vi "Get Item Icon.vi"(8 "error in (no error)":errorcluster, 11 "VI in":refnum<class "VI.lvclass">) -> (0 "error out":errorcluster, 3 "VI out":refnum<class "VI.lvclass">)   [LabVIEW 2020, in "VI Properties Editor.lvlib" / "VI.lvclass"]
doc: "Gets the icon for <B>VI in</B>."
uses:
  VI.lvclass
  VI.lvclass/VI.ctl
  <vilib>/LabVIEW Icon API/lv_icon/Controls/Alignment.ctl
  <vilib>/LabVIEW Icon API/lv_icon/Controls/Font.ctl
  <vilib>/LabVIEW Icon API/lv_icon/Controls/BodyText.ctl
  <vilib>/LabVIEW Icon API/lv_icon/lv_icon.lvlib
  <vilib>/LabVIEW Icon API/LabVIEW Icon API.lvlib
  VI Properties Editor.lvlib
panel:
  in  "Localized string template":string="Template"
  in  "Localied string text":string="Text"
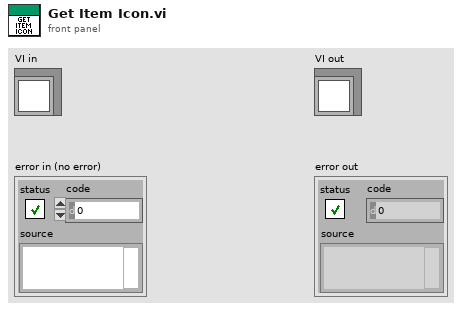
[diagram p1: front panel]
types:
  T1 = typedef "Font.ctl" = string
  T2 = typedef "BodyText.ctl" = cluster{"Line 1 text":string, "Line 2 text":string, "Line 3 text":string, "Line 4 text":string, "Line 1 color":u32, "Line 2 color":u32, "Line 3 color":u32, "Line 4 color":u32, "Body Text Spec":cluster{"Font":T1, "Alignment":T3, "Size":u8}, "Center text vertically":bool, "Capitalize Text":bool}
  T3 = typedef "Alignment.ctl" = u16
  T4 = typedef "LabVIEW Icon Stored Information.ctl" = cluster{"Text Visible?":bool, "Text Opacity":u8, "Templ Visible?":bool, "Templ Opacity":u8, "Relative Path from 1 to 2":path, "Image":picture, "All User Layers":refnum<class "Layer.lvclass">[], "Body Text":T2}
  T5 = typedef "imagedata.ctl" = cluster{"image type":i32, "image depth":i32, "image":u8[], "mask":u8[], "colors":u32[], "Rectangle":cluster{"left":i16, "top":i16, "right":i16, "bottom":i16}}
  T6 = typedef "Layer.ctl" = cluster{"LayerIcon":picture, "LayerName":string, "Opacity":u8, "Visibility?":bool}
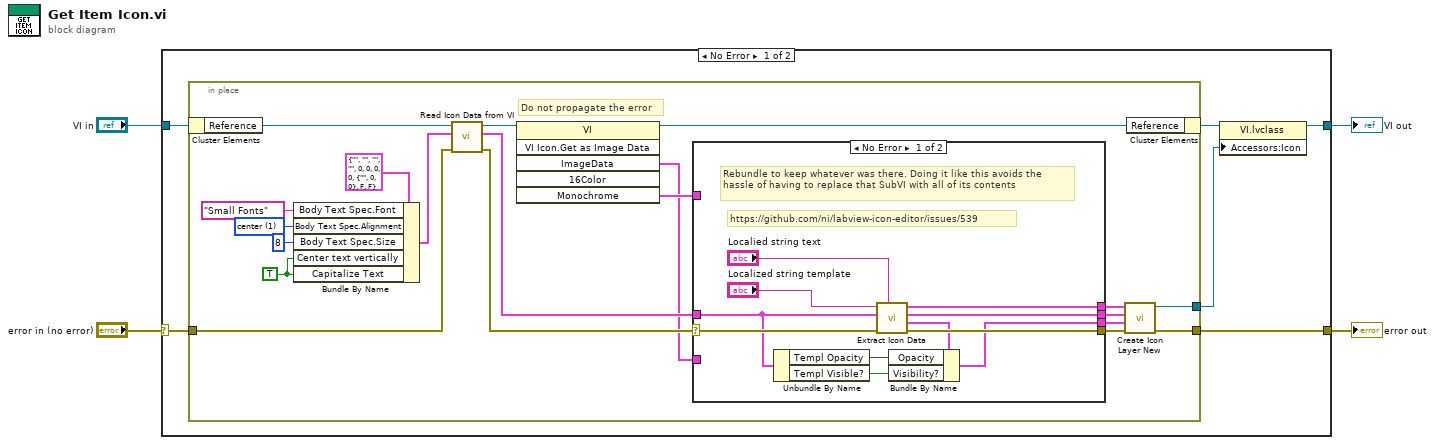
[diagram p0: block diagram]
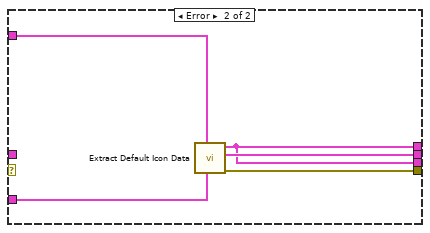
[diagram p2: hidden frame]
diagram:
  n1 = case shown="No Error" "error in (no error)" {
    selector: "error in (no error)" -> [w9 w46]
    tunnel: "VI in" -> [w10 w47]
    tunnel: [w8 w46] -> w2
    tunnel: [w5 w47] -> w1
    frame No Error {
      n2 = in-place {
        in-place-border: w9 -> [w28]
        in-place-border: [w18] -> w8
        in-place-border: [w17] -> w6
        w12 = TRUE ("Center text vertically")
        w14 = T3 1 items=["left", "center", "right"] ("Body Text Spec.Alignment")
        # "Do not propagate the error"
        n3 = in-place-cluster #1(w10) -> ("Reference"=w30:refnum<vi>)
        n4 = Bundle By Name(cluster=T2 {"Line 1 text"="", "Line 2 text"="", "Line 3 text"="", "Line 4 text"="", "Line 1 color"=0, "Line 2 color"=0, "Line 3 color"=0, "Line 4 color"=0, "Body Text Spec"={"Font"="", "Alignment"=0, "Size"=0}, "Center text vertically"=FALSE, "Capitalize Text"=FALSE} ("Default body text"), "Body Text Spec.Font"=T1 "Small Fonts", "Body Text Spec.Alignment"=w14, "Body Text Spec.Size"=u8 8, "Center text vertically"=w12, "Capitalize Text"=w12) -> (w11:T2)
        n5 = call <vilib>:"Read Icon Data from VI.vi"("error in (no error)"=w28, "Default body text"=w11, "VI Ref in"=w30) -> ("error out"=w26:errorcluster, "Data"=w25:T4, "VI Ref out"=w27:refnum<vi>)  [unwired: 6 in]
        n6 = invoke class="VI" method="VI Icon.Get as Image Data"(reference=w27) -> (reference out=w29:refnum<vi>, "ImageData"=w23:T5, "Monochrome"=w24:T5)  [unwired: 5 in, 3 out]
        n7 = case shown="No Error" w26 {
          selector: w26 -> [w40 _]
          tunnel: [w40 w44] -> w22
          tunnel: w25 -> [w34 _]
          tunnel: [w38 w42] -> w19
          tunnel: [w37 w45] -> w20
          tunnel: [w31 w42] -> w21
          tunnel: w23 -> [_ w43]
          tunnel: w24 -> [_ w41]
          frame No Error {
            # "https://github.com/ni/labview-icon-editor/issues/539"
            # "Rebundle to keep whatever was there. Doing it like this avoids the hassle of having to replace that SubVI with all of its contents"
            n8 = Unbundle By Name(w34) -> ("Templ Opacity"=w33:u8, "Templ Visible?"=w32:bool)
            n9 = call <vilib>:"Extract Icon Data.vi"("Text layer name"="Localied string text", "Icon data in"=w34, "Template layer name"="Localized string template") -> ("Template data"=w35:T6, "Icon data out"=w37:T4, "Text data"=w38:T6)  [unwired: 5 in, 1 out]
            n10 = Bundle By Name(cluster=w35, "Opacity"=w33, "Visibility?"=w32) -> (w31:T6)
          }
          frame Error {
            n11 = call <vilib>:"Extract Default Icon Data.vi"("Color Icon"=w43, "BW Icon"=w41) -> ("error out"=w44:errorcluster, "VI Icon Data out"=w45:T4, "Default Icon Template data"=w42:T6)  [unwired: 7 in]
          }
        }
        n12 = call "Create Icon Layer New.vi"("error in (no error)"=w22, "Template data"=w21, "Icon data"=w20, "Text data"=w19) -> ("error out"=w18:errorcluster, "Icon out"=w17:refnum<class "Icon.lvclass">)  [unwired: 6 in]
        n13 = in-place-cluster #1("Reference"=w29) -> (w7:refnum<class "VI.lvclass">)
      }
      n14 = property class="VI.lvclass"(reference=w7, "Accessors:Icon"=w6) -> (reference out=w5:refnum<class "VI.lvclass">)  [unwired: 1 in, 1 out]
    }
    frame Error {
    }
  }
  "error out" <- w2
  "VI out" <- w1
